vi "RDC-Lin-Reflection_Correction.vi"(7 "Tau":dbl format="%#_6e", 10 "Measured":T1) -> (1 "Reflection Tip":cdb[](array[numeric]), 2 "Tip":T1)   [LabVIEW 2020, in "RDC-Reflection_Data_Computation.lvlib"]
doc: "Corrects the reflection of the Measured Common Format cluster with the delay Tau. Returns the tip reflection array and the Tip cluster."
uses:
  RDC-Reflection_Data_Computation.lvlib
  Reflector/RFH-common_data_format.ctl
  Reflector/RFH-Reflection_File_Handler.lvlib
panel:
  out "Reflection":dbl[][](graph)
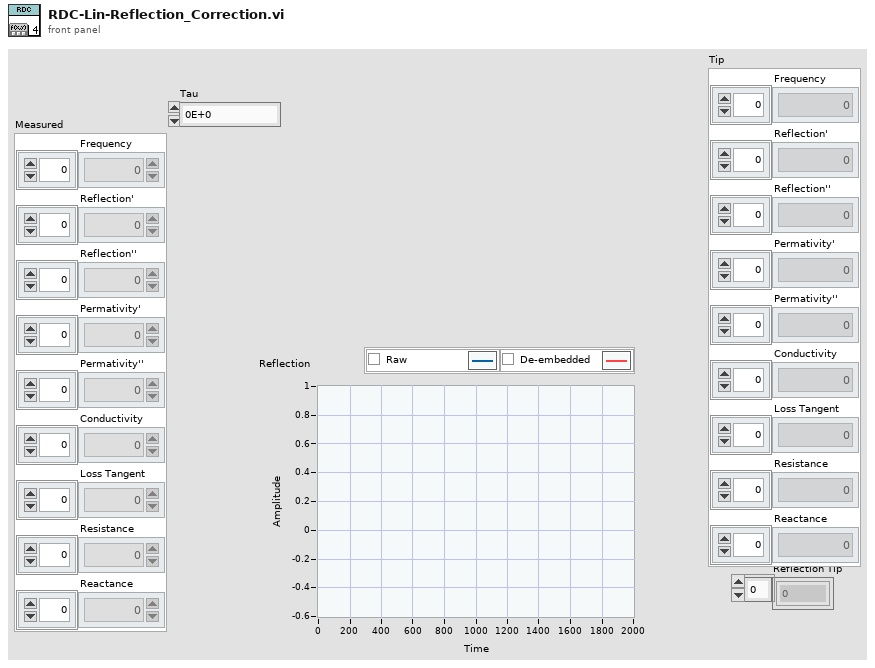
[diagram p1: front panel]
types:
  T1 = typedef "RFH-Reflection_File_Handler.lvlib/RFH-common_data_format.ctl" = cluster{"Frequency":dbl[], "Reflection'":dbl[], "Reflection''":dbl[], "Permativity'":dbl[], "Permativity''":dbl[], "Conductivity":dbl[], "Loss Tangent":dbl[], "Resistance":dbl[], "Reactance":dbl[]}
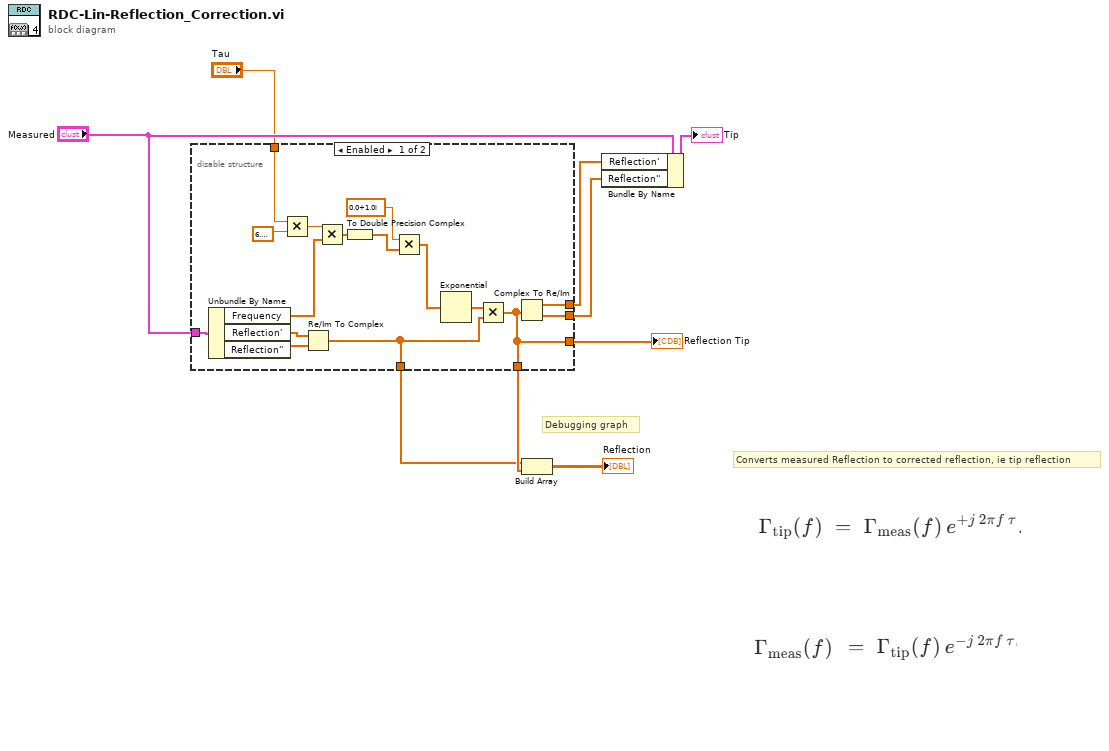
[diagram p0: block diagram]
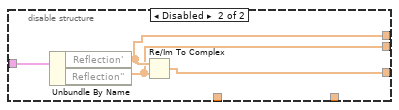
[diagram p2: hidden frame]
diagram:
  # "Debugging graph"
  # "Converts measured Reflection to corrected reflection, ie tip reflection"
  n1 = disable-structure shown="Enabled" {
    disable-tunnel: [w11 w28] -> w9
    disable-tunnel: "Measured" -> [w17 w29]
    disable-tunnel: [w14 w27] -> w6
    disable-tunnel: [w13 w26] -> w5
    disable-tunnel: "Tau" -> [w12 _]
    disable-tunnel: [w11 _] -> w2
    disable-tunnel: [w10 _] -> w1
    frame Enabled {
      n2 = Unbundle By Name(w17) -> ("Frequency"=w22:dbl[], "Reflection'"=w19:dbl[], "Reflection''"=w18:dbl[])
      n3 = Multiply(x=w12, y=6.283185307179586) -> (x*y=w23:dbl)
      n4 = Re/Im To Complex(1:w18, 2:w19) -> (0:w10:cdb[])
      n5 = Multiply(x=w23, y=w22) -> (x*y=w16:dbl[])
      n6 = To Double Precision Complex(1:w16) -> (0:w15:cdb[])
      n7 = Multiply(x=cdb 0.0+1.0i, y=w15) -> (x*y=w20:cdb[])
      n8 = Exponential(1:w20) -> (0:w25:cdb[])
      n9 = Multiply(x=w25, y=w10) -> (x*y=w11:cdb[])
      n10 = Complex To Re/Im(x + iy=w11) -> (x=w14:dbl[], y=w13:dbl[])
    }
    frame Disabled {
      n11 = Unbundle By Name(w29) -> ("Reflection'"=w27:dbl[], "Reflection''"=w26:dbl[])
      n12 = Re/Im To Complex(1:w26, 2:w27) -> (0:w28:cdb[])
    }
  }
  "Reflection Tip" <- w9
  n13 = Build Array(w1, w2) -> (→"Reflection":cdb[][])
  n14 = Bundle By Name(cluster="Measured", "Reflection'"=w6, "Reflection''"=w5) -> (→"Tip":T1)
